vi "Update Object.vi"(11 "Scene in":refnum<class "Scene.lvclass">) -> (3 "Scene out":refnum<class "Scene.lvclass">)   [LabVIEW 2020, in "Application.lvlib" / "Scene.lvclass"]
uses:
  Scene.lvclass
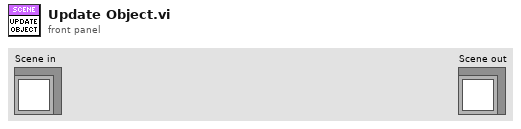
[diagram p1: front panel]
types:
  T1 = typedef "3D.lvlib/Transform.ctl" = cluster{"Position":T2, "Rotation":T2, "Scale":T2}
  T2 = typedef "3D.lvlib/Vector 3D.ctl" = cluster{"x":sgl, "y":sgl, "z":sgl}
  T3 = typedef "3D.lvlib/Object.ctl" = cluster{"Triangles":T4[], "Transform":T1, "Name":string, "Alpha Blending Enabled":bool, "Alpha":dbl, "Turntable Enabled":bool, "Material":T7}
  T4 = typedef "3D.lvlib/Triangle.ctl" = cluster{"Vertex 1":T5, "Vertex 2":T5, "Vertex 3":T5, "Alpha":dbl, "Alpha Blending Enabled":bool, "Colour":u32, "Material":T7}
  T5 = typedef "3D.lvlib/Vertex.ctl" = cluster{"Position":T2, "UV":T6, "Colour":u32}
  T6 = typedef "Raster.lvlib/UV.ctl" = cluster{"u":sgl, "v":sgl}
  T7 = typedef "3D.lvlib/Material.ctl" = cluster{"Diffuse Colour":u32, "Texture":T8}
  T8 = typedef "Raster.lvlib/Texture.ctl" = cluster{"Pixels":refnum<data-value>, "Size":T9}
  T9 = typedef "Raster.lvlib/Rectangle Dimensions.ctl" = cluster{"Width":u32, "Height":u32}
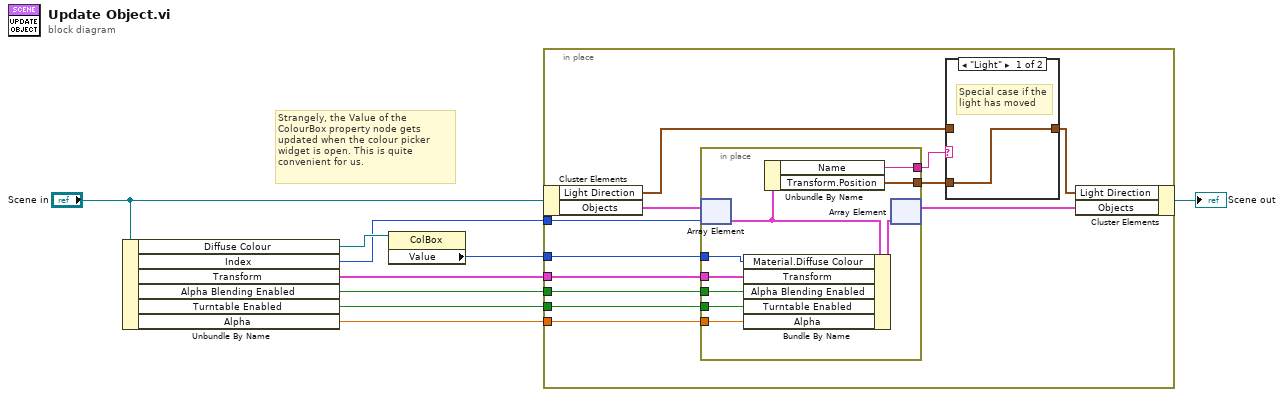
[diagram p0: block diagram]
diagram:
  # "Strangely, the Value of the ColourBox property node gets updated when the colour picker widget is open. This is quite convenient for us."
  n1 = Unbundle By Name("Scene in") -> ("Diffuse Colour"=w7:refnum<vi>, "Index"=w5:i32, "Transform"=w3:T1, "Alpha Blending Enabled"=w4:bool, "Turntable Enabled"=w2:bool, "Alpha"=w1:dbl)
  n2 = property class="ColBox"(reference=w7) -> ("Value"=w6:u32)  [unwired: 1 in, 2 out]
  n3 = in-place {
    in-place-border: w5 -> [w20]
    in-place-border: w3 -> [w18]
    in-place-border: w4 -> [w12]
    in-place-border: w6 -> [w17]
    in-place-border: w2 -> [w11]
    in-place-border: w1 -> [w10]
    n4 = in-place-cluster #1("Scene in") -> ("Light Direction"=w14:T2, "Objects"=w21:T3[])
    n5 = in-place {
      in-place-border: w18 -> [w31]
      in-place-border: w17 -> [w30]
      in-place-border: [w28] -> w16
      in-place-border: [w27] -> w13
      in-place-border: w12 -> [w26]
      in-place-border: w11 -> [w25]
      in-place-border: w10 -> [w24]
      n6 = in-place-array #2(w21, w20) -> (w29:T3)
      n7 = Bundle By Name(cluster=w29, "Material.Diffuse Colour"=w30, "Transform"=w31, "Alpha Blending Enabled"=w26, "Turntable Enabled"=w25, "Alpha"=w24) -> (w32:T3)
      n8 = Unbundle By Name(w29) -> ("Name"=w28:string, "Transform.Position"=w27:T2)
      n9 = in-place-array #2(w32) -> (w19:T3[])  [unwired: 1 out]
    }
    n10 = case shown="\"Light\"" w16 {
      tunnel: [w22 w23] -> w15
      tunnel: w14 -> [_ w23]
      tunnel: w13 -> [w22 _]
      frame "Light" {
        # "Special case if the light has moved"
      }
      frame Default {
      }
    }
    n11 = in-place-cluster #1("Light Direction"=w15, "Objects"=w19) -> (→"Scene out":refnum<class "Scene.lvclass">)
  }
